vi "SP SP - get subsubpanel.vi"(8 "error in (no error)":errorcluster, 10 "subpanel":string, 11 "subsubpanel":string) -> (0 "error out":errorcluster, 1 "references":T1, 2 "SubSubPanel found":bool, 3 "SubSubPanel VI":refnum<vi>)   [LabVIEW 2020, in "ui-testing.lvlib"]
uses:
  ui-testing.lvlib
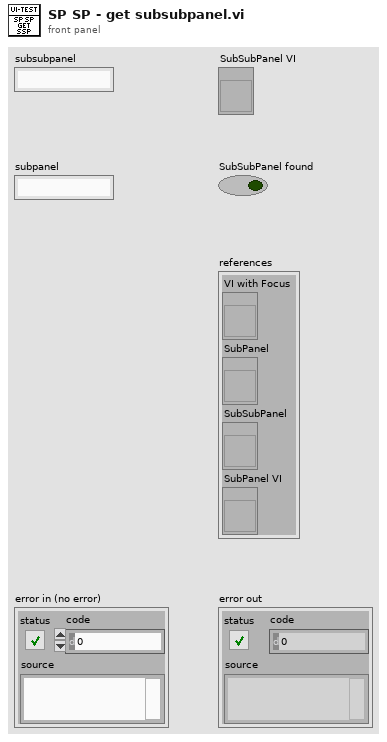
[diagram p1: front panel]
types:
  T1 = cluster{"VI with Focus":refnum<vi>, "SubPanel":refnum<vi>, "SubSubPanel":refnum<vi>, "SubPanel VI":refnum<vi>}
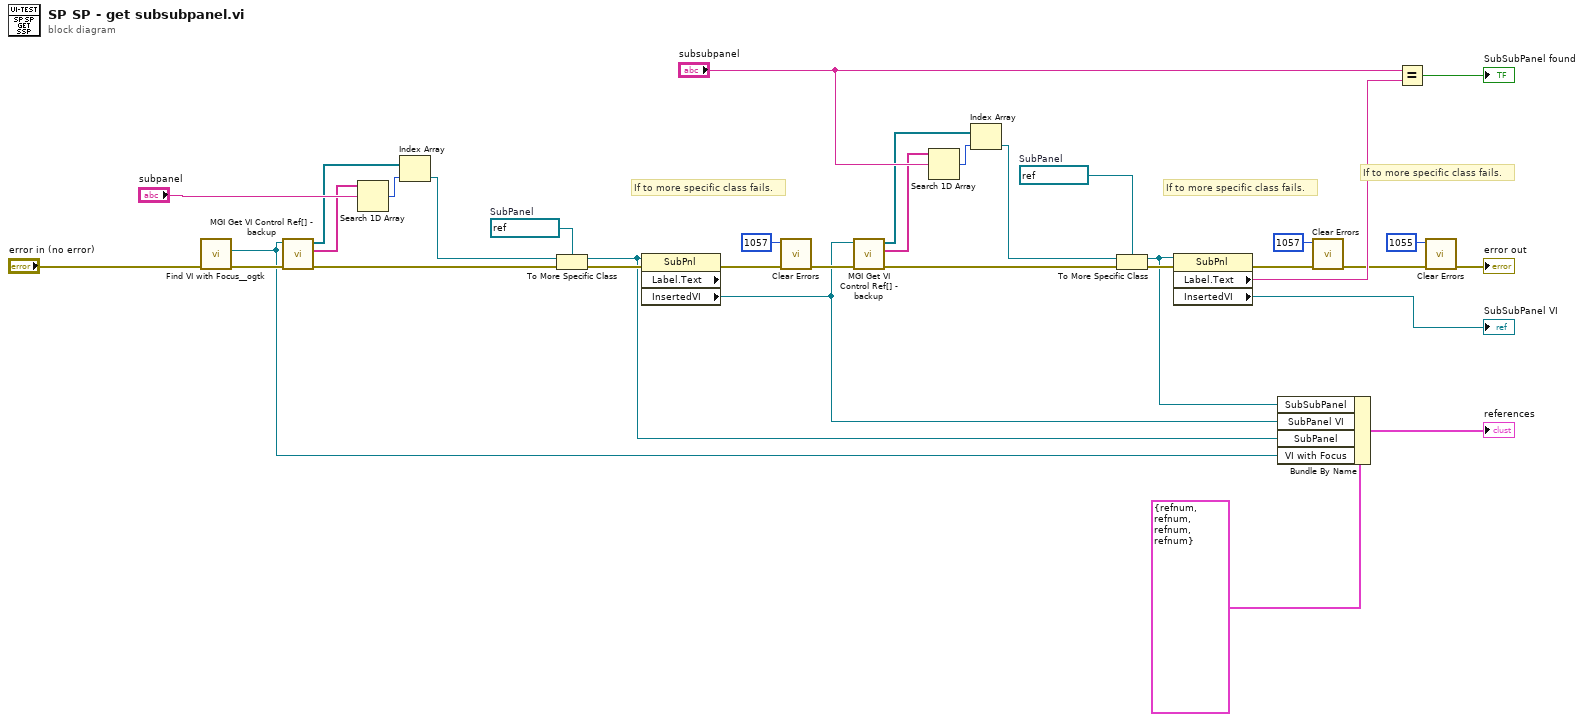
[diagram p0: block diagram]
diagram:
  w22 = refnum<vi> refnum  # SubPanel
  w19 = refnum<vi> refnum  # SubPanel
  # "If to more specific class fails."
  # "If to more specific class fails."
  # "If to more specific class fails."
  n1 = call <userlib>:"Find VI with Focus__ogtk.vi"("error in"="error in (no error)") -> ("error out"=w14:errorcluster, "VI with Focus"=w8:refnum<vi>)  [unwired: 6 in, 3 out]
  n2 = call "MGI Get VI Control Ref[] - backup.vi"("error in"=w14, "VI (Caller)"=w8) -> ("error out"=w20:errorcluster, "Control Label Chain[i]"=w11:string[], "Control[i]"=w12:refnum<vi>[])  [unwired: 6 in, 1 out]
  n3 = Search 1D Array(1D array=w11, element="subpanel") -> (index of element=w13:i32)  [unwired: 1 in]
  n4 = Index Array(array=w12, index=w13) -> (element=w21:refnum<vi>)
  n5 = To More Specific Class(target class=w19, reference=w21, error in=w20) -> (specific class reference=w6:refnum<vi>, error out=w18:errorcluster)
  n6 = property class="SubPnl" props=["Label", "Text", "InsertedVI"](reference=w6, error in=w18) -> (error out=w16:errorcluster, "InsertedVI"=w5:refnum<vi>)  [unwired: 2 out]
  n7 = call <vilib>:"Clear Errors.vi"("error in (no error)"=w16, "specific error code to clear (0: all)"=1057) -> ("error out"=w32:errorcluster)  [unwired: 4 in, 1 out]
  n8 = call "MGI Get VI Control Ref[] - backup.vi"("error in"=w32, "VI (Caller)"=w5) -> ("error out"=w33:errorcluster, "Control Label Chain[i]"=w29:string[], "Control[i]"=w30:refnum<vi>[])  [unwired: 6 in, 1 out]
  n9 = Search 1D Array(1D array=w29, element="subsubpanel") -> (index of element=w31:i32)  [unwired: 1 in]
  n10 = Index Array(array=w30, index=w31) -> (element=w34:refnum<vi>)
  n11 = To More Specific Class(target class=w22, reference=w34, error in=w33) -> (specific class reference=w7:refnum<vi>, error out=w23:errorcluster)
  n12 = property class="SubPnl"(reference=w7, error in=w23) -> (error out=w27:errorcluster, "Label.Text"=w24:string, "InsertedVI"=→"SubSubPanel VI":refnum<vi>)  [unwired: 1 out]
  n13 = Bundle By Name(cluster=T1 {"VI with Focus"=refnum, "SubPanel"=refnum, "SubSubPanel"=refnum, "SubPanel VI"=refnum}, "SubSubPanel"=w7, "SubPanel VI"=w5, "SubPanel"=w6, "VI with Focus"=w8) -> (→"references":T1)
  n14 = call <vilib>:"Clear Errors.vi"("error in (no error)"=w27, "specific error code to clear (0: all)"=1057) -> ("error out"=w3:errorcluster)  [unwired: 4 in, 1 out]
  n15 = Equal?(x="subsubpanel", y=w24) -> (x = y?=→"SubSubPanel found":bool)
  n16 = call <vilib>:"Clear Errors.vi"("error in (no error)"=w3, "specific error code to clear (0: all)"=1055) -> ("error out"=→"error out":errorcluster)  [unwired: 4 in, 1 out]
